vi "RemoteVI Server Setup.vi"(0 "VI":refnum<vi>, 1 "view only?":bool, 5 "fps":dbl=20.0, 9 "window":u64, 11 "error in":errorcluster) -> (2 "origin":cluster{"x":i32, "y":i32}, 3 "period":dbl, 4 "hello":string, 6 "html":string, 7 "VI name":string, 8 "geo":T1, 10 "hWnd":u64, 12 "VI out":refnum<vi>, 13 "window out":u64, 14 "mode":string, 15 "error out":errorcluster)   [LabVIEW 2020, in "RemoteVI.lvlib"]
doc: "(VI, or a window of any process when window is not 0.) What the server loop needs before its first iteration: hello (the greeting frames with the name of VI, RemoteVI Greeting.vi), html (the web client, RemoteVI Index HTML.vi), the panel geometry, window handle and origin of the panel inside the frame (RemoteVI Get Panel Geometry.vi) and period = 1000 / fps ms. error out carries error in and the error of reading the VI name."
uses:
  RemoteVI.lvlib
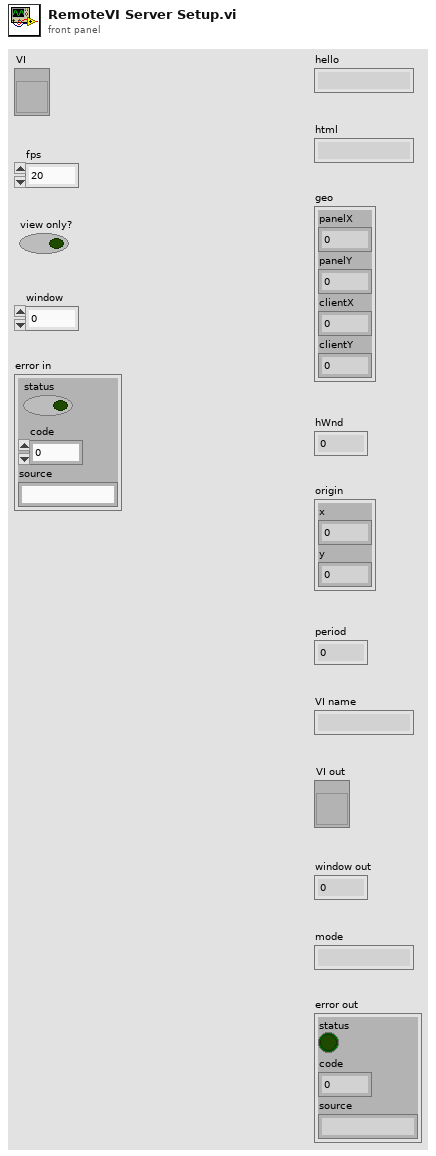
[diagram p1: front panel]
types:
  T1 = cluster{"panelX":i32, "panelY":i32, "clientX":i32, "clientY":i32}
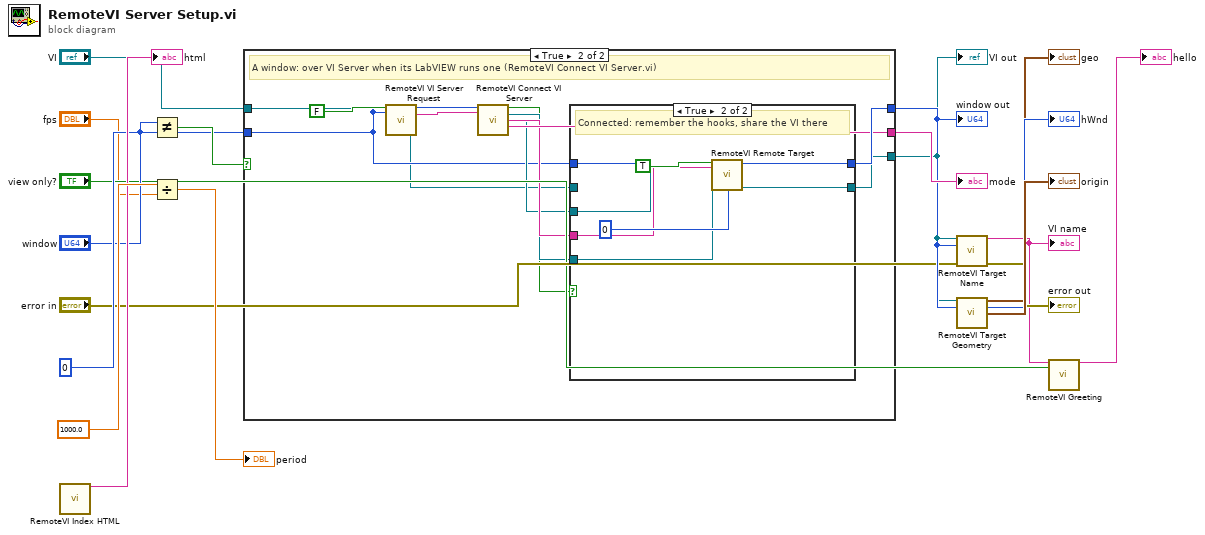
[diagram p0: block diagram]
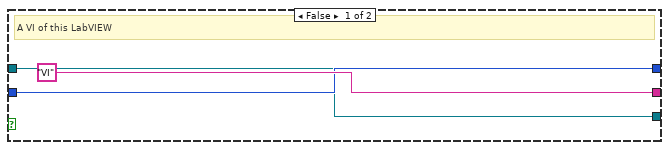
[diagram p2: hidden frame]
diagram:
  n1 = call "RemoteVI Index HTML.vi"() -> ("html"=→"html":string)  [unwired: 14 in, 1 out]
  n2 = Not Equal?(x="window", y=u64 0) -> (x != y?=w7:bool)
  n3 = Divide(x=1000.0, y="fps") -> (x/y=→"period":dbl)
  n4 = case shown="True" w7 {
    tunnel: "VI" -> [w20 w23]
    tunnel: "window" -> [w21 w24]
    tunnel: [w21 w33] -> w9
    tunnel: ["VI" w31] -> w10
    tunnel: [w20 w32] -> w8
    frame False {
      # "A VI of this LabVIEW"
    }
    frame True {
      # "A window: over VI Server when its LabVIEW runs one (RemoteVI Connect VI Server.vi)"
      n5 = call "RemoteVI VI Server Request.vi"("put?"=FALSE, "hWnd"=w24) -> ("address out"=w26:string)  [unwired: 11 in, 2 out]
      n6 = call "RemoteVI Connect VI Server.vi"("window"=w24, "address"=w26) -> ("connected?"=w27:bool, "VI"=w28:refnum<vi>, "hooks"=w29:refnum<vi>, "VI name"=w30:string, "mode"=w31:string)  [unwired: 9 in]
      n7 = case shown="True" w27 {
        tunnel: [w34 u64 0] -> w33
        tunnel: w24 -> [w34 w36]
        tunnel: w23 -> [w35 _]
        tunnel: w29 -> [_ w37]
        tunnel: w30 -> [_ w38]
        tunnel: w28 -> [_ w39]
        tunnel: [w35 w39] -> w32
        frame False {
          # "Window only"
        }
        frame True {
          # "Connected: remember the hooks, share the VI there"
          n8 = call "RemoteVI Remote Target.vi"("put?"=TRUE, "hWnd"=w36, "hooks"=w37, "VI name"=w38) -> ()  [unwired: 9 in, 3 out]
        }
      }
    }
  }
  "VI out" <- w8
  "window out" <- w9
  "mode" <- w10
  n9 = call "RemoteVI Target Name.vi"("VI"=w8, "window"=w9, "error in"="error in") -> ("name"=w11:string, "error out"=→"error out":errorcluster)  [unwired: 11 in]
  "VI name" <- w11
  n10 = call "RemoteVI Target Geometry.vi"("VI"=w8, "window"=w9) -> ("geo"=→"geo":T1, "hWnd"=→"hWnd":u64, "origin"=→"origin":cluster{"x":i32, "y":i32})  [unwired: 10 in, 1 out]
  n11 = call "RemoteVI Greeting.vi"("VI name"=w11, "view only?"="view only?") -> ("hello"=→"hello":string)  [unwired: 13 in]
